vi "TrapProfile_Execute.vi"(4 "Initialize":bool, 5 "Max Speed":dbl format="%20.4f", 6 "TimePeriod":dbl=0.02 format="%20.4f", 7 "Max Accel":dbl format="%20.4f", 8 "CurrentVelocity":dbl format="%20.4f", 9 "CurrentPosition":dbl format="%20.4f", 10 "GoalVelocity":dbl format="%20.4f", 11 "GoalPosition":dbl format="%20.4f") -> (0 "TimeFinished":bool, 1 "EstTimeLeft":dbl, 2 "VelocityDmd":dbl, 3 "PositionDmd":dbl)   [LabVIEW 2019, in "Trajectory_Library.lvlib"]
doc: "Convience, single call, LabVIEW function. Creates and calculates a Trapezoid Profile. Call this routine periodically to calculate the newest output for the provided inputs. \n\nOne use of a Trapezoid Profile is to calculate a velocity SP (Setpoint) for a position movement so that the velocity SP creates a trapezoid shape to allow for smoother operation and reduced overshoot. \n \nInputs:\n - Max Speed -- Maximum allowable speed\n - Max Accel -- Maximum allowable acceleration\n - Goal Position -- Deisred final position\n - Goal Velocity -- Desired velocity when goal position is reached. (Might often be zero.)\n - Current Position -- Current position (This could be a measured value.)\n - Current Velocity -- Current velocity (This could be a measured value.)\n - TimePeriod -- Period between calls in seconds.\n - Initialize -- If TRUE, the Goal values are reset to the inputs and the initial position and velocity are set to the current position and velocity.\n\nOutputs:\n - PositionDmd -- Current position demand (This could be used to calculate position error, or used in control.)\n - VelocityDmd -- Current velocity demand. (This could be used as a setpoint to drive an actuator or motor.)\n - EstTimeLeft -- Estimated time remaining until goal is achieved.\n - TimeFinished -- The goal should have been reached because the estimated calculated time has expired."
uses:
  Trajectory_Library.lvlib
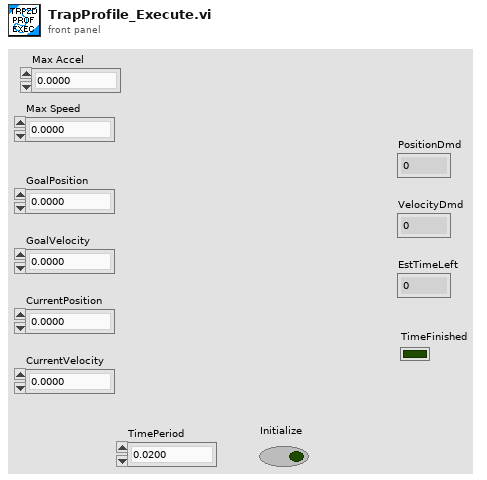
[diagram p1: front panel]
types:
  T1 = typedef "WPILib_Math.lvlib/TRAPEZOID_PROFILE_STATE.ctl" = cluster{"Position":dbl, "Velocity":dbl}
  T2 = typedef "WPILib_Math.lvlib/TRAPEZOID_PROFILE_CONSTRAINT.ctl" = cluster{"MaxVelocity":dbl, "MaxAcceleration":dbl}
  T3 = typedef "WPILib_Math.lvlib/TRAPEZOID_PROFILE.ctl" = cluster{"EndAccel":dbl, "EndFullSpeed":dbl, "EndDecel":dbl, "Direction":i32, "Constraints":T2, "Initial":T1, "Goal":T1}
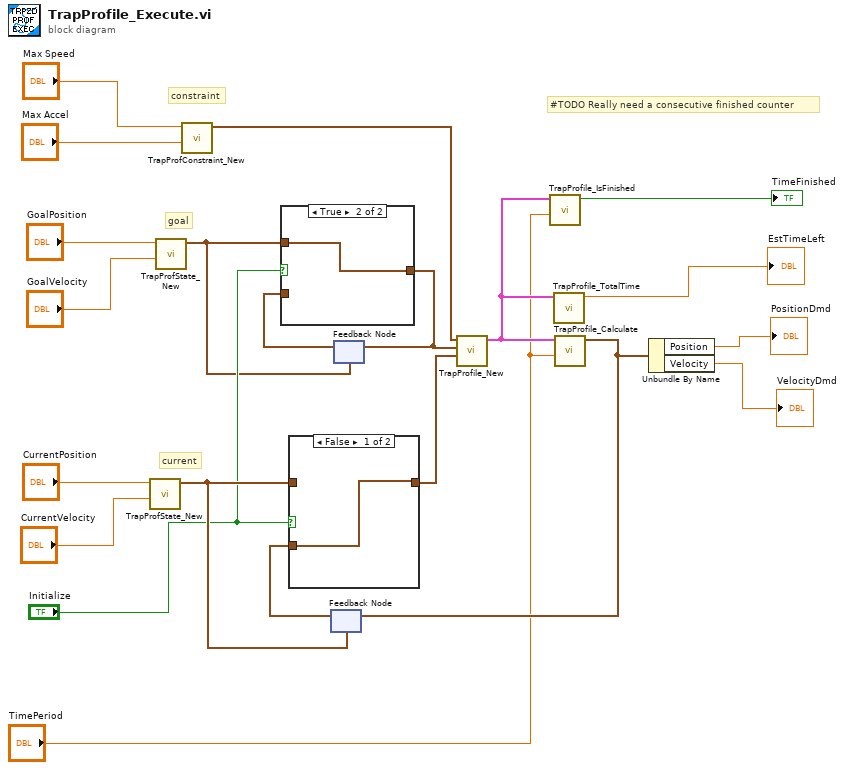
[diagram p0: block diagram]
diagram:
  # "#TODO Really need a consecutive finished counter"
  # "current"
  # "goal"
  # "constraint"
  n1 = call "TrapProfState_New.vi"("Velocity"="CurrentVelocity", "Position"="CurrentPosition") -> ("TRAPEZOID_PROFILE_STATE"=w10:T1)  [unwired: 9 in]
  n2 = call "TrapProfState_New.vi"("Velocity"="GoalVelocity", "Position"="GoalPosition") -> ("TRAPEZOID_PROFILE_STATE"=w3:T1)  [unwired: 9 in]
  n3 = call "TrapProfConstraint_New.vi"("Max Accel"="Max Accel", "Max Speed (M/S)"="Max Speed") -> ("TRAPEZOID_PROFILE_CONSTRAINT"=w21:T2)  [unwired: 9 in]
  n4 = feedback #1(w10) -> (w8:T1)
  n5 = case shown="False" "Initialize" {
    tunnel: w10 -> [_ w23]
    tunnel: [w22 w23] -> w11
    tunnel: w8 -> [w22 _]
    frame False {
    }
    frame True {
    }
  }
  n6 = feedback #2(w3) -> (w2:T1)
  n7 = case shown="True" "Initialize" {
    tunnel: w3 -> [_ w25]
    tunnel: [w24 w25] -> w4
    tunnel: w2 -> [w24 _]
    frame False {
    }
    frame True {
    }
  }
  n8 = feedback-in #2(w4) -> ()
  n9 = call "TrapProfile_New.vi"("Initial"=w11, "Goal"=w4, "Constraints"=w21) -> ("TRAPEZOID_PROFILE"=w7:T3)  [unwired: 8 in]
  n10 = call "TrapProfile_IsFinished.vi"("Time"="TimePeriod", "TRAPEZOID_PROFILE"=w7) -> ("Finished"=→"TimeFinished":bool)  [unwired: 9 in]
  n11 = call "TrapProfile_TotalTime.vi"("TRAPEZOID_PROFILE"=w7) -> ("TotalTime"=→"EstTimeLeft":dbl)  [unwired: 10 in]
  n12 = call "TrapProfile_Calculate.vi"("Time"="TimePeriod", "TRAPEZOID_PROFILE"=w7) -> ("State"=w9:T1)  [unwired: 9 in]
  n13 = feedback-in #1(w9) -> ()
  n14 = Unbundle By Name(w9) -> ("Position"=→"PositionDmd":dbl, "Velocity"=→"VelocityDmd":dbl)
